vi "Configure Measurement.vi"(8 "error in (no error)":errorcluster, 10 "Window Handle":i32, 11 "Config File Path":path=path "TestStand.ini") -> (0 "error out":errorcluster, 1 "Show UI?":bool, 2 "Device Names":string[](array[string]), 3 "Measurement Name":string, 4 "Array of Device Configuration":refnum<class "HW Configuration.lvclass">[](array[class]), 6 "Measurement Actor.lvlib:Step Configuration.lvclass":refnum<class "Step Configuration.lvclass">)   [LabVIEW 2017, in "Measurement Setup Controller.lvlib" / "Measurement Setup.lvclass"]
uses:
  Measurement Setup.lvclass
  <userlib>/Common Components/Hardware/HW Config/HW Configuration.lvclass
  <userlib>/Common Components/Measurement Actor/Configuration/Step Configuration.lvclass
  <userlib>/Common Components/Msmt Configuration/Controller Configuration.lvclass
  C:/Program Files (x86)/National Instruments/LabVIEW 2017/user.lib/Configuration Dialog Actor/Configuration.lvclass
  UI/Measurement Setup UI.lvclass
  C:/Program Files (x86)/National Instruments/LabVIEW 2017/user.lib/Common Components/User Interface/UI.lvclass
  <vilib>/ActorFramework/LastAck/Last Ack.lvclass
  C:/Program Files (x86)/National Instruments/LabVIEW 2017/user.lib/Common Components/Controller/Controller.lvclass
  C:/Program Files (x86)/National Instruments/LabVIEW 2017/vi.lib/ActorFramework/Actor/Actor.lvclass
  <vilib>/ActorFramework/Message Queue/Message Queue.lvclass/Message Queue.ctl
  UI/Measurement Setup UI.lvclass/Measurement Setup UI.ctl
  <vilib>/ActorFramework/Message Dequeuer/Message Dequeuer.lvclass/Message Dequeuer.ctl
  <vilib>/ActorFramework/LastAck/Last Ack.lvclass/Last Ack.ctl
  Measurement Setup.lvclass/Measurement Setup.ctl
  Measurement Data/Measurement Data.lvclass/Measurement Data.ctl
  <vilib>/ActorFramework/Message Priority Queue/Priority Dequeue.vi
  Measurement Data/Measurement Data.lvclass
  <vilib>/ActorFramework/Message Queue/Message Queue.lvclass
  <vilib>/ActorFramework/Message Dequeuer/Message Dequeuer.lvclass
  <vilib>/ActorFramework/Actor/Actor.lvclass
  <userlib>/Common Components/Controller/Controller.lvclass
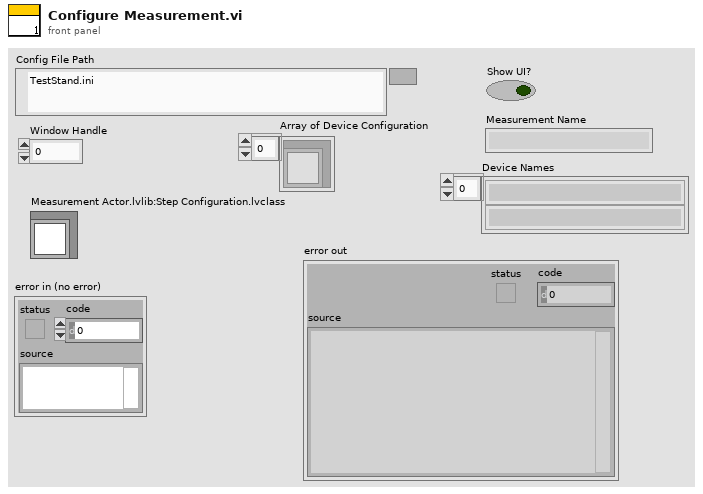
[diagram p1: front panel]
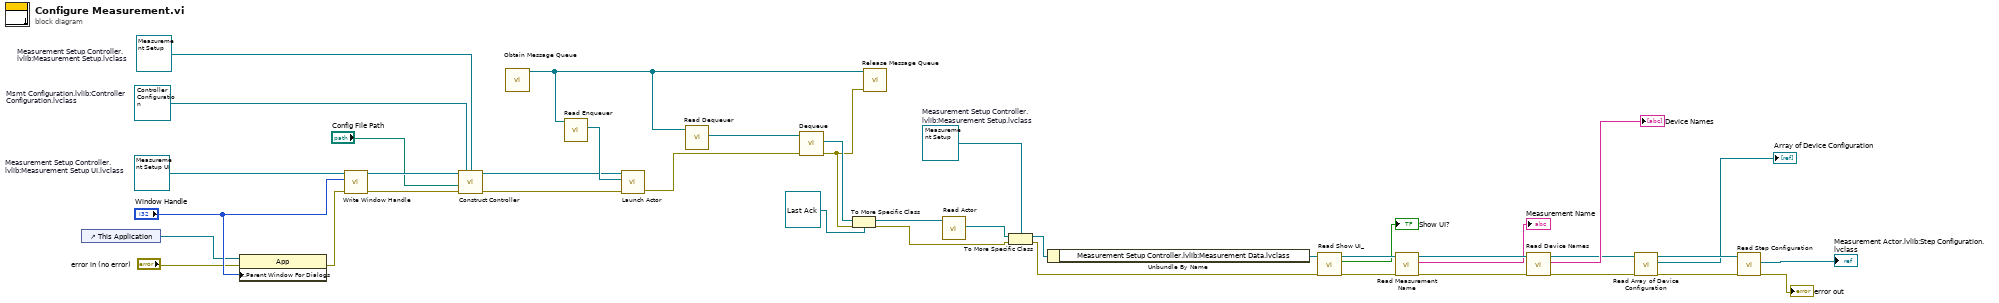
[diagram p0: block diagram]
diagram:
  w33 = refnum<class "Measurement Setup.lvclass"> refnum  # Measurement Setup Controller.lvlib:Measurement Setup.lvclass
  w40 = refnum<class "Measurement Setup UI.lvclass"> refnum  # Measurement Setup Controller.lvlib:Measurement Setup UI.lvclass
  w14 = refnum<class "Measurement Setup.lvclass"> refnum  # Measurement Setup Controller.lvlib:Measurement Setup.lvclass
  w13 = refnum<class "Controller Configuration.lvclass"> refnum  # Msmt Configuration.lvlib:Controller Configuration.lvclass
  n1 = control-ref of="This Application"() -> (w19:refnum<vi>)
  n2 = property class="App"(reference=w19, error in="error in (no error)", "Application:Parent Window For Dialogs"="Window Handle") -> (error out=w18:errorcluster)  [unwired: 1 out]
  n3 = call "Write Window Handle.vi"("error in (no error)"=w18, "Window Handle"="Window Handle", "Measurement Setup UI in"=w40) -> ("error out"=w11:errorcluster, "Measurement Setup UI out"=w15:refnum<class "Measurement Setup UI.lvclass">)  [unwired: 7 in]
  n4 = call <userlib>:"Construct Controller.vi"("UI.lvclass"=w15, "error in (no error)"=w11, "Root Path"="Config File Path", "Configuration.lvlib:Configuration.lvclass"=w13, "Controller Actor.lvlib:Controller.lvclass"=w14) -> ("error out"=w9:errorcluster, "Controller Actor.lvlib:Controller.lvclass 2"=w8:refnum<class "Measurement Setup.lvclass">)  [unwired: 4 in, 1 out]
  n5 = call <vilib>:"Obtain Message Queue.vi"() -> ("Message Queue"=w39:refnum<class "Message Queue.lvclass">)  [unwired: 10 in, 1 out]
  n6 = call <vilib>:"Read Enqueuer.vi"("Message Queue"=w39) -> ("Message Enqueuer"=w17:refnum<class "Message Enqueuer.lvclass">)  [unwired: 10 in]
  n7 = call <vilib>:"Launch Actor.vi"("error in (no error)"=w9, "Actor-to-Caller Enqueuer"=w17, "Actor"=w8) -> ("error out"=w16:errorcluster)  [unwired: 7 in, 1 out]
  n8 = call <vilib>:"Read Dequeuer.vi"("Message Queue"=w39) -> ("Message Dequeuer"=w38:refnum<class "Message Dequeuer.lvclass">)  [unwired: 10 in]
  n9 = call <vilib>:"Dequeue.vi"("error in (no error)"=w16, "Message Dequeuer in"=w38) -> ("error out"=w21:errorcluster, "Message"=w37:refnum<class "Message.lvclass">)  [unwired: 5 in, 3 out]
  n10 = To More Specific Class(target class=refnum<class "Last Ack.lvclass"> refnum ("Last Ack"), reference=w37, error in=w21) -> (specific class reference=w35:refnum<class "Last Ack.lvclass">, error out=w25:errorcluster)
  n11 = call <vilib>:"Release Message Queue.vi"("error in (no error)"=w21, "Message Queue"=w39) -> ()  [unwired: 8 in, 2 out]
  n12 = call <vilib>:"Read Actor.vi"("Last Ack"=w35) -> ("Actor"=w34:refnum<class "Actor.lvclass">)  [unwired: 10 in]
  n13 = To More Specific Class(target class=w33, reference=w34, error in=w25) -> (specific class reference=w32:refnum<class "Measurement Setup.lvclass">, error out=w28:errorcluster)
  n14 = Unbundle By Name(w32) -> ("Measurement Setup Controller.lvlib:Measurement Data.lvclass"=w31:refnum<class "Measurement Data.lvclass">)
  n15 = call "Read Show UI_.vi"("error in (no error)"=w28, "Measurement Data in"=w31) -> ("error out"=w27:errorcluster, "Show UI?"=→"Show UI?":bool, "Measurement Data out"=w30:refnum<class "Measurement Data.lvclass">)  [unwired: 7 in]
  n16 = call "Read Measurement Name.vi"("error in (no error)"=w27, "Measurement Data in"=w30) -> ("error out"=w26:errorcluster, "Measurement Name"=→"Measurement Name":string, "Measurement Data out"=w29:refnum<class "Measurement Data.lvclass">)  [unwired: 7 in]
  n17 = call "Read Device Names.vi"("error in (no error)"=w26, "Measurement Data in"=w29) -> ("error out"=w3:errorcluster, "Device Names"=→"Device Names":string[], "Measurement Data out"=w7:refnum<class "Measurement Data.lvclass">)  [unwired: 7 in]
  n18 = call "Read Array of Device Configuration.vi"("error in (no error)"=w3, "Measurement Data in"=w7) -> ("error out"=w2:errorcluster, "Array of Device Configuration"=→"Array of Device Configuration":refnum<class "HW Configuration.lvclass">[], "Measurement Data out"=w6:refnum<class "Measurement Data.lvclass">)  [unwired: 7 in]
  n19 = call "Read Step Configuration.vi"("error in (no error)"=w2, "Measurement Data in"=w6) -> ("error out"=→"error out":errorcluster, "Measurement Actor.lvlib:Step Configuration.lvclass"=→"Measurement Actor.lvlib:Step Configuration.lvclass":refnum<class "Step Configuration.lvclass">)  [unwired: 7 in, 1 out]
